vi "SetTestv2NoRbac.vi"() -> ()   [LabVIEW 2017]
uses:
  <vilib>/httpClient/POSTBuffer.vi
  <vilib>/httpClient/LabVIEWHTTPClient.lvlib
  <vilib>/Analysis/NI_AALBase.lvlib
panel:
  out "body":string
  out "standard deviation":dbl format="%0.2f"
  out "mean":dbl format="%0.2f"
  out "error out":errorcluster
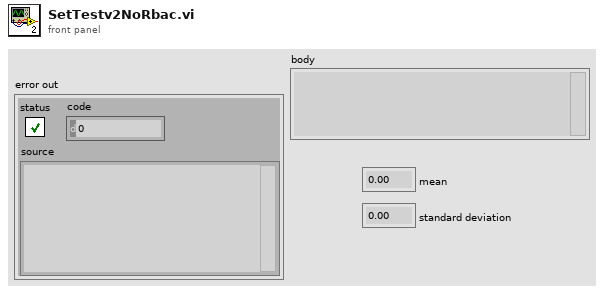
[diagram p1: front panel]
types:
  T1 = cluster{"req_action":string, "selector":string, "req_lang":string, "device":string, "type_descriptor":i16[]}
  T2 = cluster{"dbl_field":dbl, "string_field":string, "long_field":i64, "int_array_field":i32[]}
  T3 = typedef "LabVIEWHTTPClient.lvlib/ClientHandle.ctl" = refnum<k1>
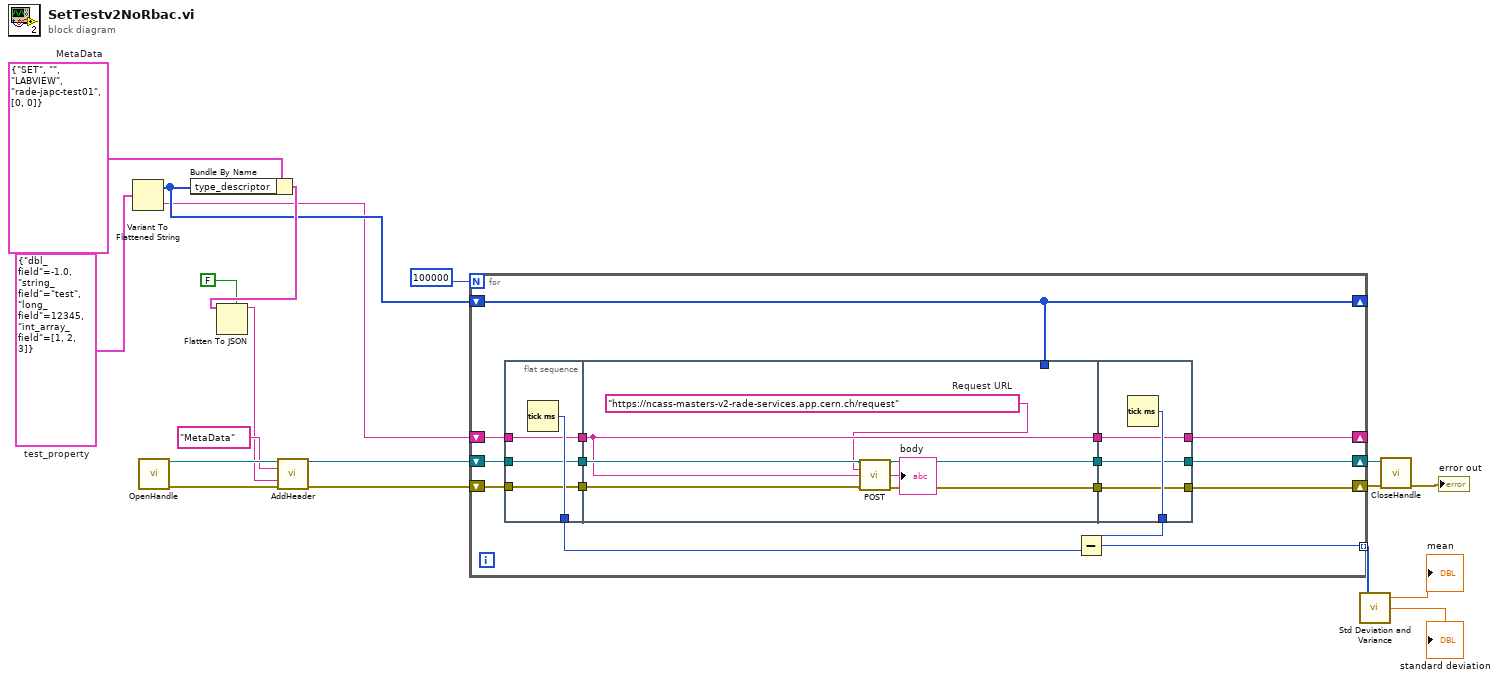
[diagram p0: block diagram]
diagram:
  w7 = T1 {"req_action"="SET", "selector"="", "req_lang"="LABVIEW", "device"="rade-japc-test01", "type_descriptor"=[0, 0]}  # MetaData
  w3 = T2 {"dbl_field"=-1.0, "string_field"="test", "long_field"=12345, "int_array_field"=[1, 2, 3]}  # test_property
  n1 = Variant To Flattened String(Variant=w3) -> (data string=w1:string, 1:w2:i16[])
  n2 = call <vilib>:"OpenHandle.vi"() -> ("client handle out"=w17:T3, "error out"=w18:errorcluster)  [unwired: 14 in]
  n3 = Bundle By Name(cluster=w7, "type_descriptor"=w2) -> (w6:T1)
  n4 = Flatten To JSON(enable LabVIEW extensions? (T)=FALSE, anything=w6) -> (JSON string=w4:string)  [unwired: 1 in, 1 out]
  n5 = call <vilib>:"AddHeader.vi"("client handle"=w17, "header"="MetaData", "value"=w4, "error in (no error)"=w18) -> ("client handle out"=w9:T3, "error out"=w8:errorcluster)  [unwired: 10 in]
  n6 = for {
    N: 100000 -> [_]
    shift-right: [w35] -> _
    shift-left: w2 -> [w35]
    tunnel: [w30] -> w12 mode=indexing
    shift-right: [w31] -> w14
    shift-left: w9 -> [w28]
    shift-right: [w20] -> w13
    shift-left: w8 -> [w26]
    shift-right: [w22] -> _
    shift-left: w1 -> [w24]
    n7 = flat-sequence {
      tunnel: [w39] -> w34
      tunnel: [w38] -> w29
      tunnel: w28 -> [w38]
      tunnel: [w37] -> w27
      tunnel: w26 -> [w37]
      tunnel: [w36] -> w25
      tunnel: w24 -> [w36]
      tunnel: w35 -> [_]
      tunnel: [w44] -> w32
      tunnel: w29 -> [w46]
      tunnel: w27 -> [w45]
      tunnel: w25 -> [w43]
      tunnel: [w43] -> w23
      tunnel: [w42] -> w21
      tunnel: [w50] -> w33
      tunnel: [w49] -> w31
      tunnel: w32 -> [w49]
      tunnel: w23 -> [w48]
      tunnel: [w48] -> w22
      tunnel: [w47] -> w20
      tunnel: w21 -> [w47]
      frame #0 {
        n8 = Tick Count (ms)() -> (millisecond timer value=w39:u32)
      }
      frame #1 {
        w40 = "https://ncass-masters-v2-rade-services.app.cern.ch/request"  # Request URL
        n9 = call-poly <vilib>:"POST.vi"("client handle"=w46, "url"=w40, "buffer"=w43, "error in (no error)"=w45) -> ("client handle out"=w44:T3, "body"=→"body":string, "error out"=w42:errorcluster)  [unwired: 8 in, 1 out]
      }
      frame #2 {
        n10 = Tick Count (ms)() -> (millisecond timer value=w50:u32)
      }
    }
    n11 = Subtract(x=w33, y=w34) -> (x-y=w30:u32)
  }
  n12 = call <vilib>:"Std Deviation and Variance.vi"("X"=w12) -> ("mean"=→"mean":dbl, "standard deviation"=→"standard deviation":dbl)  [unwired: 1 in, 1 out]
  n13 = call <vilib>:"CloseHandle.vi"("client handle"=w14, "error in (no error)"=w13) -> ("error out"=→"error out":errorcluster)  [unwired: 13 in]
